vi "SimulatorGlobalOscilloscope.vi"() -> ()   [LabVIEW 2014]
panel:
  in  "Timeout":u16
  in  "Telemetry from LabviewOscilloscope":string
  in  "Telecommand to LabviewOscilloscope":string
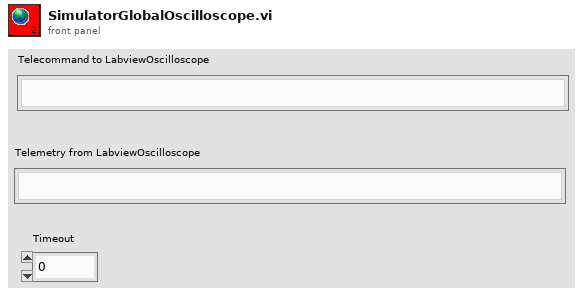
[diagram p1: front panel]
diagram:
